vi "Host - Find Slave Path.vi"(8 "error in (no error)":errorcluster, 11 "Item Ref in":T1 format="%.0x") -> (0 "error out":errorcluster, 1 "Target IP Address":string, 2 "Slave Ref":string, 3 "Item Ref out":T1=18446744073709551615 format="%.0x")   [LabVIEW 2020, in "SEECD System Explorer.lvlib"]
uses:
  SEECD System Explorer.lvlib
  <vilib>/NI VeriStand/Custom Device API/Custom Device Item Ref.ctl
  <vilib>/NI VeriStand/Custom Device API/Custom Device API.lvlib
  Scripting/Scan Engine Scripting.lvlib
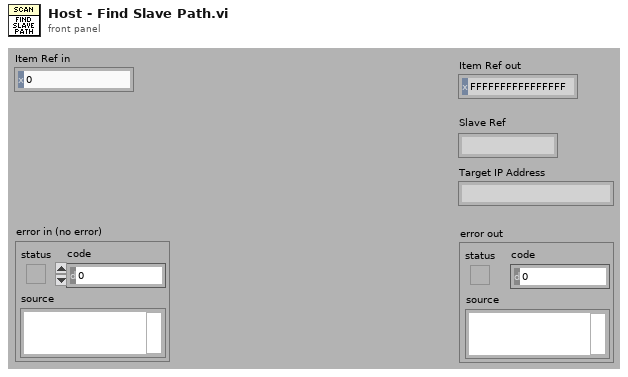
[diagram p1: front panel]
types:
  T1 = typedef "Custom Device API.lvlib/Custom Device Item Ref.ctl" = u64
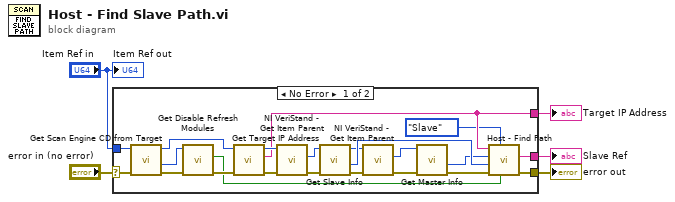
[diagram p0: block diagram]
diagram:
  n1 = case shown="No Error" "error in (no error)" {
    selector: "error in (no error)" -> [w12 w28]
    tunnel: "Item Ref in" -> [w11 _]
    tunnel: [w18 w28] -> w4
    tunnel: [w15 _] -> w2
    tunnel: [w13 _] -> w1
    frame No Error {
      n2 = call "Get Scan Engine CD from Target.vi"("error in"=w12, "Item Ref in"=w11) -> ("error out"=w8:errorcluster, "scan engine custom device ref"=w10:T1, "Item Ref out"=w9:T1)  [unwired: 7 in]
      n3 = call "Get Disable Refresh Modules.vi"("error in"=w8, "scan engine custom device ref in"=w10) -> ("error out"=w7:errorcluster, "disable refresh modules"=w6:bool)  [unwired: 7 in, 1 out]
      n4 = call "Get Target IP Address.vi"("error in"=w7, "Item Ref in"=w9) -> ("error out"=w17:errorcluster, "Target IP Address"=w15:string, "Item Ref out"=w16:T1)  [unwired: 7 in]
      n5 = call <vilib>:"NI VeriStand - Get Item Parent.vi"("error in (no error)"=w17, "Item Ref in"=w16) -> ("error out"=w20:errorcluster, "Parent Ref"=w19:T1)  [unwired: 6 in, 2 out]
      n6 = call "Get Slave Info.vi"("error in (no error)"=w20, "Item Ref in"=w19) -> ("error out"=w22:errorcluster, "Slave #"=w27:u16, "Item Ref out"=w21:T1)  [unwired: 4 in, 3 out]
      n7 = call <vilib>:"NI VeriStand - Get Item Parent.vi"("error in (no error)"=w22, "Item Ref in"=w21) -> ("error out"=w24:errorcluster, "Parent Ref"=w23:T1)  [unwired: 6 in, 2 out]
      n8 = call "Get Master Info.vi"("error in (no error)"=w24, "Item Ref in"=w23) -> ("error out"=w25:errorcluster, "Master #"=w26:u32)  [unwired: 6 in, 2 out]
      n9 = call "Host - Find Path.vi"("Disable Refresh Modules"=w6, "Type"=enum16{"Slave", "Master"}."Slave", "error in (no error)"=w25, "Slave Index"=w27, "Master Index"=w26, "serverName"=w15) -> ("error out"=w18:errorcluster, "Path"=w13:string)  [unwired: 4 in]
    }
    frame Error {
    }
  }
  "error out" <- w4
  "Target IP Address" <- w2
  "Slave Ref" <- w1
  "Item Ref out" <- "Item Ref in"
